vi "compare pkg versions server vs client.vi"(8 "error in (no error)":errorcluster) -> (0 "error out":errorcluster, 1 "Jl Server state out":T4, 3 "LVServer_version":T1, 4 "return code":u8, 5 "timeout?":bool, 6 "detailed error info":T2)   [LabVIEW 2018, in "LV2Julia_core.lvlib"]
uses:
  LV2Julia_core.lvlib
  Server or client state.ctl
  detailed error info.ctl
  StackFrame.ctl
  VersionNumber.ctl
  ef5b6aa2-77b9-48db-bc29-60677fa9782d.vi
  ef5b6aa2-77b9-48db-bc29-60677fa9782d.vi/1ed83875-98c1-444a-beff-8cbe044ed12a.vi
  ef5b6aa2-77b9-48db-bc29-60677fa9782d.vi/1ed83875-98c1-444a-beff-8cbe044ed12a.vi/b17fa786-f84d-4754-b57b-5b75e84dca16.vi
  ef5b6aa2-77b9-48db-bc29-60677fa9782d.vi/1ed83875-98c1-444a-beff-8cbe044ed12a.vi/cb4745a3-3287-482a-b76d-441bec049f49.vi
  ef5b6aa2-77b9-48db-bc29-60677fa9782d.vi/1ed83875-98c1-444a-beff-8cbe044ed12a.vi/42f9ddad-de74-4f5c-ab45-70883ec7d1c8.vi
  packages versions global.vi
  check ID validity.vi
  bindata_descr to JSON.vi
  check cluster field names.vi
  concat JSON.vi
  build request.vi
  REQ full lifecycle.vi
  Parse server response.vi
  log jl exceptions.vi
  <vilib>/Utility/error.llb/Error Cluster From Error Code.vi
  <vilib>/ErrorRing/Error Ring.xnode
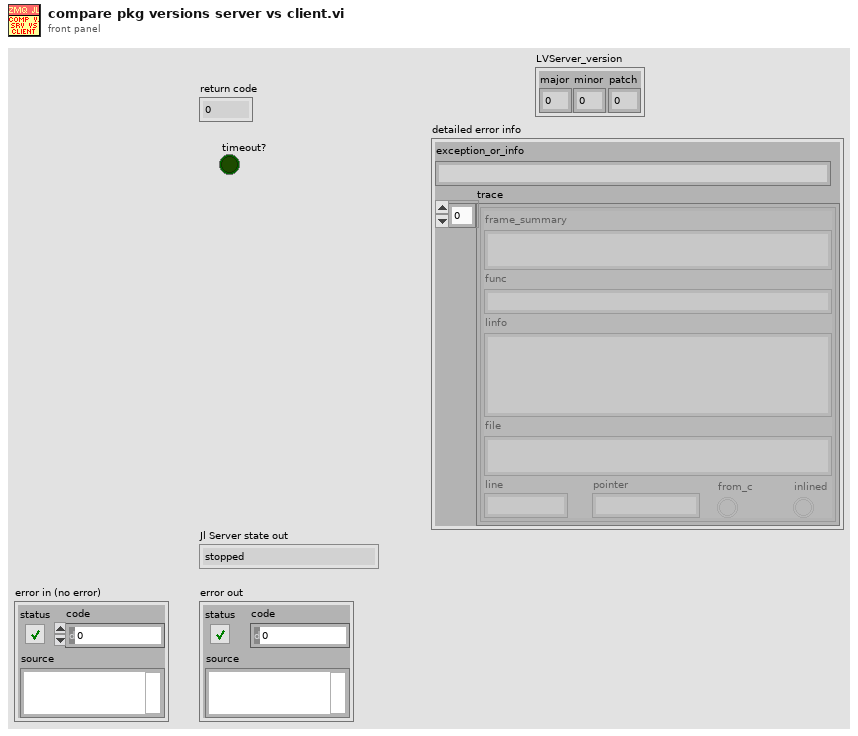
[diagram p1: front panel]
types:
  T1 = typedef "LV2Julia_core.lvlib/VersionNumber.ctl" = cluster{"major":u16, "minor":u16, "patch":u16}
  T2 = typedef "LV2Julia_core.lvlib/detailed error info.ctl" = cluster{"exception_or_info":string, "trace":T3[]}
  T3 = typedef "LV2Julia_core.lvlib/StackFrame.ctl" = cluster{"frame_summary":string, "func":string, "linfo":string, "file":string, "line":i32, "pointer":u64, "from_c":bool, "inlined":bool}
  T4 = typedef "LV2Julia_core.lvlib/Server or client state.ctl" = enum16{"stopped", "running", "unknown"}
  T5 = cluster{"LV_v":T1, "LVServer_current":T1, "LVServer_min":T1}
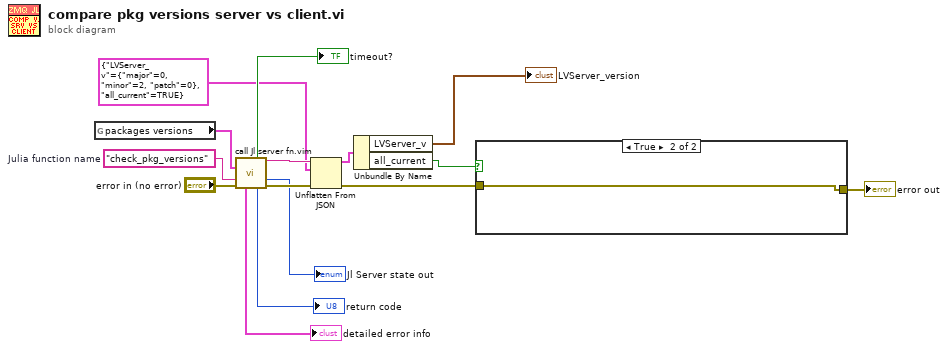
[diagram p0: block diagram]
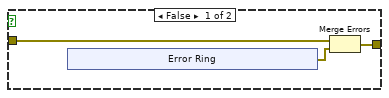
[diagram p2: hidden frame]
diagram:
  w6 = "check_pkg_versions"  # Julia function name
  n1 = global read "packages versions global.vi" "packages versions"() -> (w5:T5)
  n2 = call "call Jl server fn.vim"("Arguments 2"=w5, "fun2call"=w6, "error in (no error)"="error in (no error)") -> ("timeout?"=→"timeout?":bool, "JSON received"=w12:string, "Jl Server state out"=→"Jl Server state out":T4, "detailed error info"=→"detailed error info":T2, "return code"=→"return code":u8, "error out"=w11:errorcluster)  [unwired: 6 in, 1 out]
  n3 = Unflatten From JSON(JSON string=w12, type and defaults=cluster{"LVServer_v":T1, "all_current":bool} {"LVServer_v"={"major"=0, "minor"=2, "patch"=0}, "all_current"=TRUE}, error in (no error)=w11) -> (value=w3:cluster{"LVServer_v":T1, "all_current":bool}, error out=w14:errorcluster)  [unwired: 4 in]
  n4 = Unbundle By Name(w3) -> ("LVServer_v"=→"LVServer_version":T1, "all_current"=w2:bool)
  n5 = case shown="True" w2 {
    tunnel: [w18 w24] -> w15
    tunnel: w14 -> [w17 w24]
    frame False {
      n6 = xnode "Error Ring"() -> ("error out"=w16:errorcluster)
      n7 = Merge Errors(w17, w16) -> (w18:errorcluster)
    }
    frame True {
    }
  }
  "error out" <- w15
